vi "FP Close Path.vi"() -> ()   [LabVIEW 2020]
doc: "Dev helper: closes the front panel of the VI at path (Front Panel Window:Open = FALSE)."
panel:
  out "error out":errorcluster
  in  "path":path
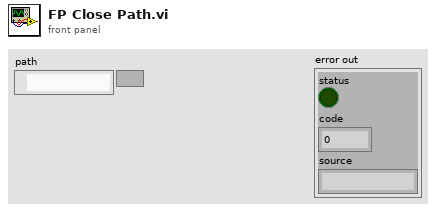
[diagram p1: front panel]
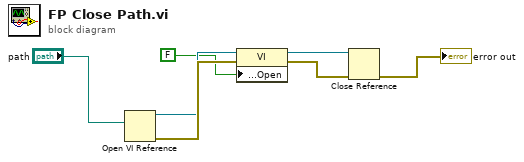
[diagram p0: block diagram]
diagram:
  n1 = Open VI Reference(vi path="path") -> (vi reference=w3:refnum<vi>, error out=w4:errorcluster)  [unwired: 5 in]
  n2 = property class="VI"(reference=w3, error in=w4, "Front Panel Window:Open"=FALSE) -> (reference out=w5:refnum<vi>, error out=w6:errorcluster)
  n3 = Close Reference(reference=w5, error in (no error)=w6) -> (error out=→"error out":errorcluster)
